vi "CreateWithCFG.vi"(8 "error in (no error)":errorcluster, 10 "Configuration":refnum<class "Configuration.lvclass">, 11 "object in":refnum<class "Channel.lvclass">) -> (0 "error out":errorcluster, 3 "object out":refnum<class "Channel.lvclass">)   [LabVIEW 2021, in "Channel.lvlib" / "Channel.lvclass"]
doc: "Creates the Channel with its configuration"
uses:
  Channel.lvclass
  Configuration_class/Configuration.lvclass
  Channel.lvclass/Channel.ctl
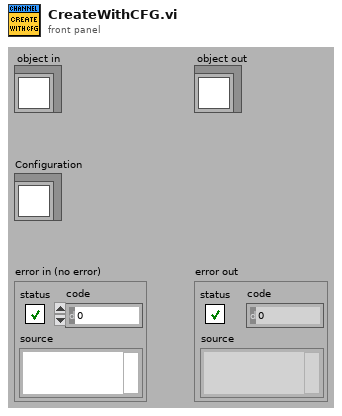
[diagram p1: front panel]
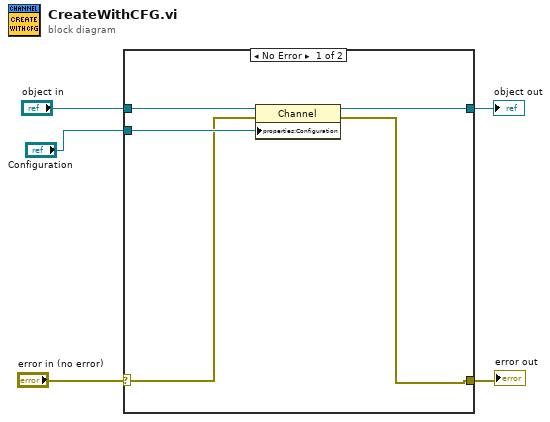
[diagram p0: block diagram]
diagram:
  n1 = case shown="No Error" "error in (no error)" {
    selector: "error in (no error)" -> [w7 w12]
    tunnel: [w6 w12] -> w4
    tunnel: [w9 w11] -> w2
    tunnel: "object in" -> [w10 w11]
    tunnel: "Configuration" -> [w8 _]
    frame No Error {
      n2 = property class="Channel"(reference=w10, error in=w7, "properties:Configuration"=w8) -> (reference out=w9:refnum<class "Channel.lvclass">, error out=w6:errorcluster)
    }
    frame Error {
    }
  }
  "error out" <- w4
  "object out" <- w2
